vi "JSON Array Size.vi"(8 "error in (no error)":errorcluster, 11 "JSON Tree In (JSON Array)":variant) -> (0 "error out":errorcluster, 2 "Array Size":i32, 3 "JSON Tree Passthrough (JSON Array)":variant)   [LabVIEW 2014, in "i3-json.lvlib"]
doc: "Returns the size of a JSON array"
uses:
  i3-json.lvlib
  JSON Types/JSON Type.ctl
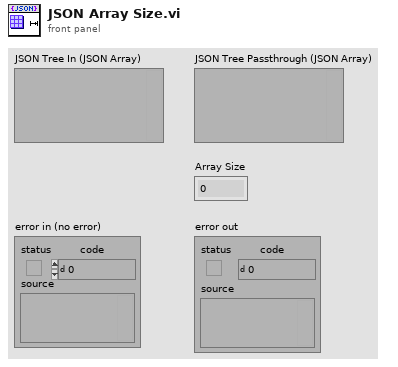
[diagram p1: front panel]
types:
  T1 = typedef "i3-json.lvlib/JSON Type.ctl" = enum8{"JSON Compatible", "JSON Array", "JSON Object", "JSON Null", "Double", "String", "Boolean", "Unknown"}
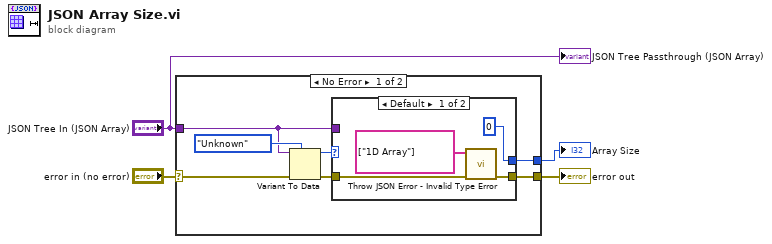
[diagram p0: block diagram]
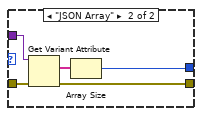
[diagram p2: hidden frame]
diagram:
  n1 = case shown="No Error" "error in (no error)" {
    selector: "error in (no error)" -> [w11 w21]
    tunnel: [w6 w21] -> w3
    tunnel: "JSON Tree In (JSON Array)" -> [w7 _]
    tunnel: [w5 _] -> w1
    frame No Error {
      n2 = Variant To Data(error in=w11, type=JSON_Type."Unknown" ("JSON Type"), Variant=w7) -> (data=w9:T1, error out=w8:errorcluster)
      n3 = case shown="Default" w9 {
        tunnel: w8 -> [w14 w20]
        tunnel: w7 -> [_ w19]
        tunnel: [w13 w18] -> w6
        tunnel: [0 w16] -> w5
        frame Default {
          n4 = call "Throw JSON Error - Invalid Type Error.vi"("error in (no error)"=w14, "Valid Types"=string[] ["1D Array"]) -> ("error out"=w13:errorcluster)  [unwired: 9 in]
        }
        frame "JSON Array" {
          n5 = Get Variant Attribute(Variant=w19, error in=w20) -> (names=w17:string[], error out=w18:errorcluster)  [unwired: 2 in, 2 out]
          n6 = Array Size(array=w17) -> (size(s)=w16:i32)
        }
      }
    }
    frame Error {
    }
  }
  "error out" <- w3
  "Array Size" <- w1
  "JSON Tree Passthrough (JSON Array)" <- "JSON Tree In (JSON Array)"
